vi "labview.vi"() -> ()   [LabVIEW 2025]
panel:
  out "Thermometer":dbl(slide) scale=0.0..100.0
  out "Gauge 2":dbl(knob) scale=0.0..4.0
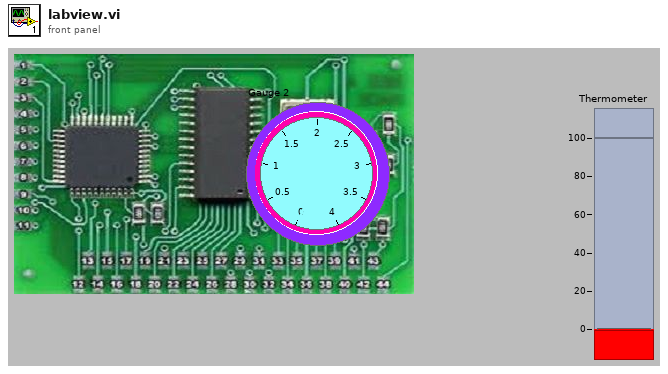
[diagram p1: front panel]
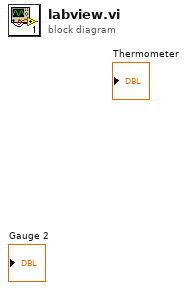
[diagram p0: block diagram]
diagram:
